vi "VIH Project - Container - Product Info.vi"(7 "cmd (get)":enum16{"get", "set"}(ring), 11 "Product Info in":T1) -> (3 "Product Info out":T1)   [LabVIEW 2014]
doc: "::: VI Helpeks :::\nCopyright (c) 2000-2026 Konstantin Shifershteyn. All rights reserved."
uses:
  _VIH HelpGen.llb/VIH HelpGen Typedef - Product Info Cluster.ctl
panel:
  # "VI Helpeks\nCopyright (c) 2012-2026 Konstantin Shifershteyn"
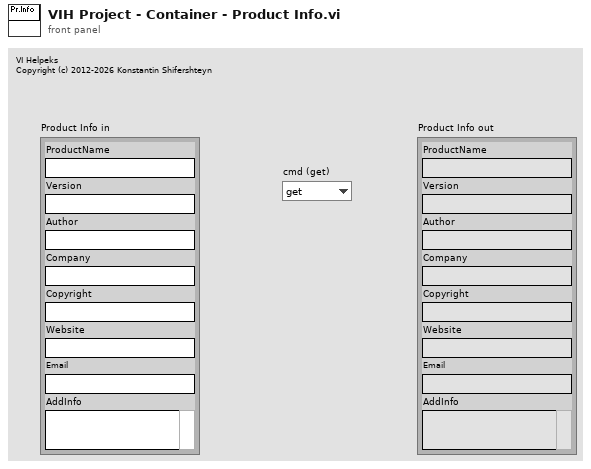
[diagram p1: front panel]
types:
  T1 = typedef "VIH HelpGen Typedef - Product Info Cluster.ctl" = cluster{"ProductName":string, "Version":string, "Author":string, "Company":string, "Copyright":string, "Website":string, "Email":string, "AddInfo":string}
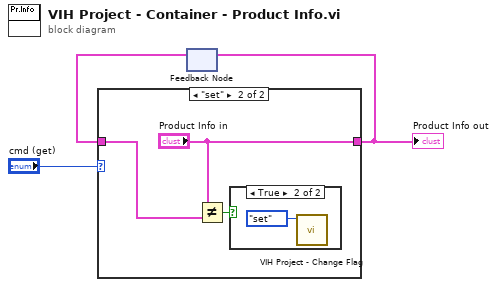
[diagram p0: block diagram]
diagram:
  n1 = feedback #1() -> (w1:T1)  [unwired: 1 in]
  n2 = case shown="\"set\"" "cmd (get)" {
    tunnel: [w4 "Product Info in"] -> w2
    tunnel: w1 -> [w4 w6]
    frame "get" {
    }
    frame "set" {
      n3 = Not Equal?(x="Product Info in", y=w6) -> (x != y?=w5:bool)
      n4 = case shown="True" w5 {
        frame False {
        }
        frame True {
          n5 = call "VIH Project - Change Flag.vi"("cmd (get)"=enum16{"get", "set", "reset"}."set") -> ()  [unwired: 9 in, 2 out]
        }
      }
    }
  }
  "Product Info out" <- w2
  n6 = feedback-in #1(w2) -> ()
